vi "PIDController_Pack_AdvLimits.vi"(4 "MinOutput":dbl=-9.9e+32, 6 "MaxOutput":dbl=9.9e+32, 9 "Continuous":bool, 10 "MinInput":dbl, 11 "MaxInput":dbl) -> (3 "Adv PID Limits":T1={"MaxInput"=0.0, "MinInput"=0.0, "Continuous"=FALSE, "MaxOutput"=9.9e+32, "MinOutput"=-9.9e+32})   [LabVIEW 2019, in "Trajectory_Library.lvlib"]
doc: "Convience function to pack individual input and output limit values into a cluster to pass to the Advanced PID controller\n\nNote -- These values are considered to be static after they are initially set. Changes during run-time may be ignored.\n\nInputs:\n\n - Max Input -- The maximum allowed input The units are the same as the Setpoint (SP) and Process variable (PV) (When both Max and Min values are 0.0, input limit checking is disabled.)\n - Min Input -- The minimum allowed input value The units are the same as the Setpoint (SP) and Process variable (PV) (When both Max and Min values are 0.0, input limit checking is disabled.)\n - Continuous -- Boolean indicating that the inputs wrap from the maximum value to the miimum value.. (Example - gyro and heading control)\n - MaxOutput -- The maximum allowed output The units are the same as the output. This is used to clamp the output and is used for anti-windup protection ( Default 9.9E+32 )\n - MinOutput -- The maximum allowed output The units are the same as the output. This is used to clamp the output and is used for anti-windup protection ( Default -9.9E+32 )\n\nOutput:\n - Adv PID Input Limits -- Cluster containing the input values"
uses:
  Trajectory_Library.lvlib
  TypeDef/PID_ADV_LIMITS.ctl
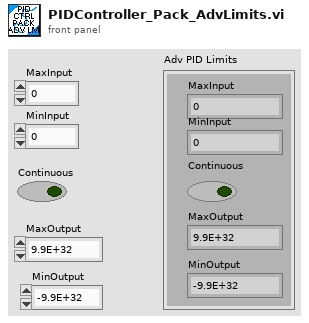
[diagram p1: front panel]
types:
  T1 = typedef "Trajectory_Library.lvlib/PID_ADV_LIMITS.ctl" = cluster{"MaxInput":dbl, "MinInput":dbl, "Continuous":bool, "MaxOutput":dbl, "MinOutput":dbl}
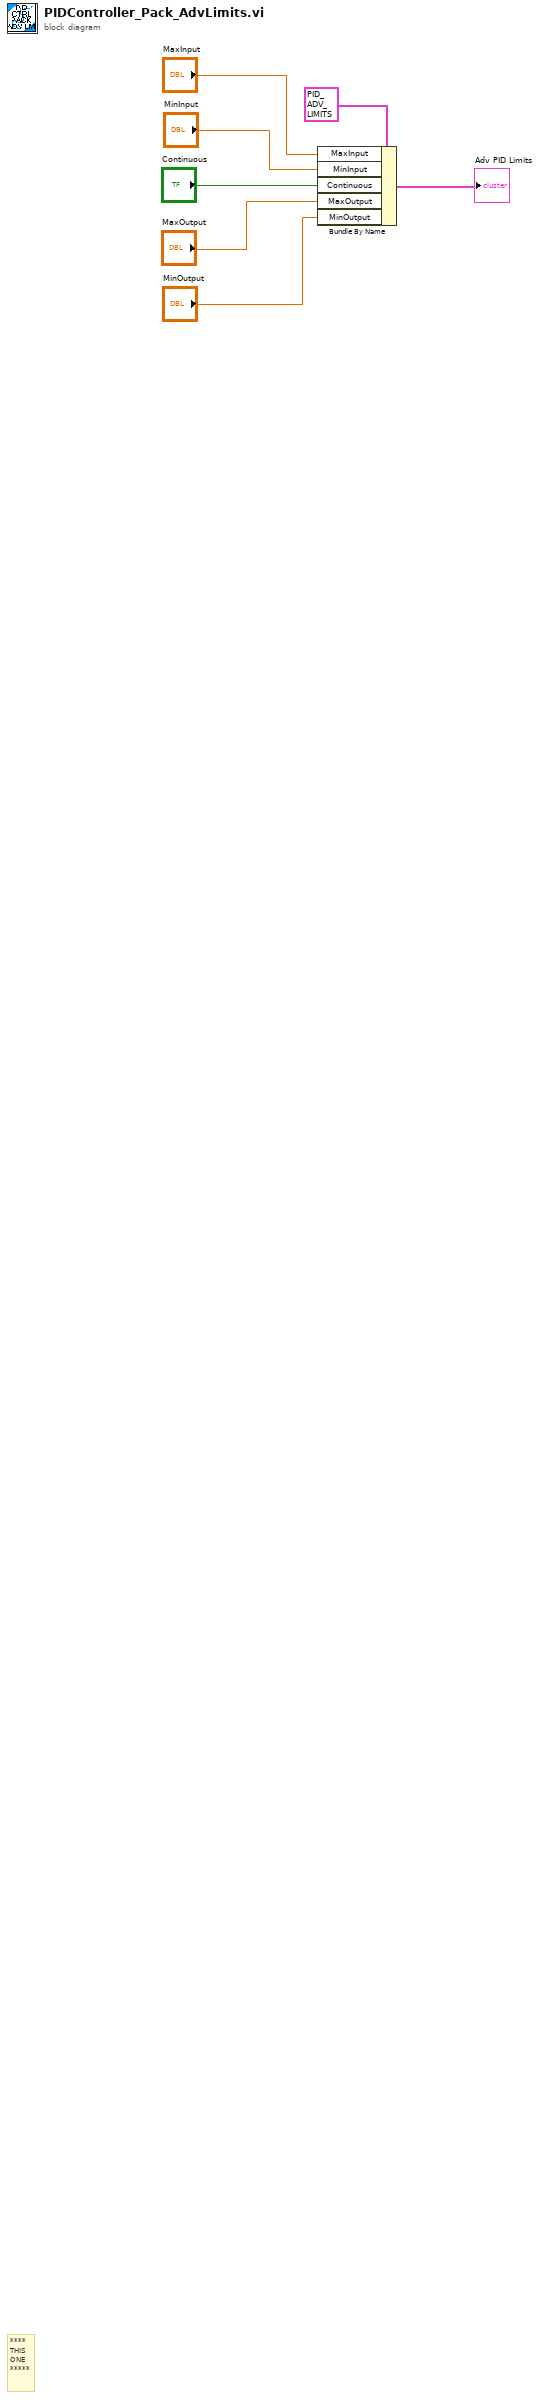
[diagram p0: block diagram]
diagram:
  # "****\nTHIS\nONE\n*****"
  n1 = Bundle By Name(cluster=T1 {"MaxInput"=0.0, "MinInput"=0.0, "Continuous"=FALSE, "MaxOutput"=9.9e+32, "MinOutput"=-9.9e+32} ("Adv PID Limits"), "MaxInput"="MaxInput", "MinInput"="MinInput", "Continuous"="Continuous", "MaxOutput"="MaxOutput", "MinOutput"="MinOutput") -> (→"Adv PID Limits":T1)
